vi "End Metric.vi"(7 "Metrics Forward":T2, 8 "error in (no error)":errorcluster, 11 "Module in":refnum<class "Module.lvclass">) -> (0 "error out":errorcluster, 3 "Module out":refnum<class "Module.lvclass">, 5 "Metrics Reverse":T1)   [LabVIEW 2020, in "Volatus.lvlib" / "Module.lvclass"]
uses:
  Module.lvclass
  Metrics Forward.ctl
  Metrics Reverse.ctl
  Module.lvclass/Module.ctl
  MessageQ/MessageQ.lvclass/MessageQ.ctl
  Forward Metric.vi
  Parent Q.vi
  MessageQ/Is Null.vi
  MessageQ/Send.vi
  <vilib>/ptbypt/NI_PtbyPt.lvlib
  Volatus.lvlib
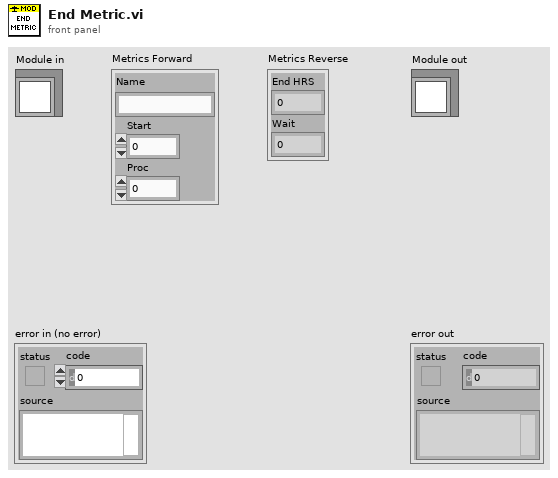
[diagram p1: front panel]
types:
  T1 = typedef "Volatus.lvlib/Metrics Reverse.ctl" = cluster{"End HRS":dbl, "Wait":dbl}
  T2 = typedef "Volatus.lvlib/Metrics Forward.ctl" = cluster{"Name":string, "Start":dbl, "Proc":dbl}
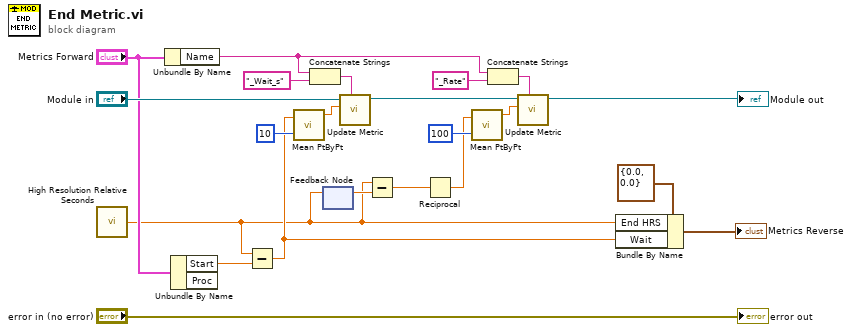
[diagram p0: block diagram]
diagram:
  n1 = call <vilib>:"High Resolution Relative Seconds.vi"() -> ("relative seconds"=w2:dbl)
  n2 = Unbundle By Name("Metrics Forward") -> ("Name"=w7:string)
  n3 = Unbundle By Name("Metrics Forward") -> ("Start"=w13:dbl)  [unwired: 1 out]
  n4 = Subtract(x=w2, y=w13) -> (x-y=w5:dbl)
  n5 = call <vilib>:"Mean PtByPt.vi"("x"=w5, "sample length"=10) -> ("mean"=w18:dbl)  [unwired: 2 in, 1 out]
  n6 = Concatenate Strings(w7, "_Wait_s" ("string")) -> (w19:string)
  n7 = feedback-in #1(w2) -> ()
  n8 = feedback #1() -> (w3:dbl)  [unwired: 1 in]
  n9 = call "Update Metric.vi"("Metric"=w19, "Value"=w18, "Module in"="Module in") -> ("Module out"=w8:refnum<class "Module.lvclass">)  [unwired: 7 in, 1 out]
  n10 = Subtract(x=w2, y=w3) -> (x-y=w1:dbl)
  n11 = Reciprocal(x=w1) -> (1/x=w4:dbl)
  n12 = call <vilib>:"Mean PtByPt.vi"("x"=w4, "sample length"=100) -> ("mean"=w9:dbl)  [unwired: 2 in, 1 out]
  n13 = Concatenate Strings(w7, "_Rate" ("string")) -> (w10:string)
  n14 = call "Update Metric.vi"("Metric"=w10, "Value"=w9, "Module in"=w8) -> ("Module out"=→"Module out":refnum<class "Module.lvclass">)  [unwired: 7 in, 1 out]
  n15 = Bundle By Name(cluster=T1 {"End HRS"=0.0, "Wait"=0.0} ("Metrics Reverse"), "End HRS"=w2, "Wait"=w5) -> (→"Metrics Reverse":T1)
  "error out" <- "error in (no error)"
